vi "Build Class Hierarchy as List.vi"(8 "error in (no error)":errorcluster, 11 "List of Class Paths":path[](array[path])) -> (0 "error out":errorcluster, 3 "List of Class Paths Out":path[](array[path]))   [LabVIEW 2012, in "Palette Generation.lvlib"]
doc: "This VI builds a list of all the parent classes of the input list of class files and returns a list of all classes in the heirarachy with the base classes firts. This ensures that when we generate the palette files, the parent class root palette file will always exist and so can be linked in."
uses:
  Palette Generation.lvlib
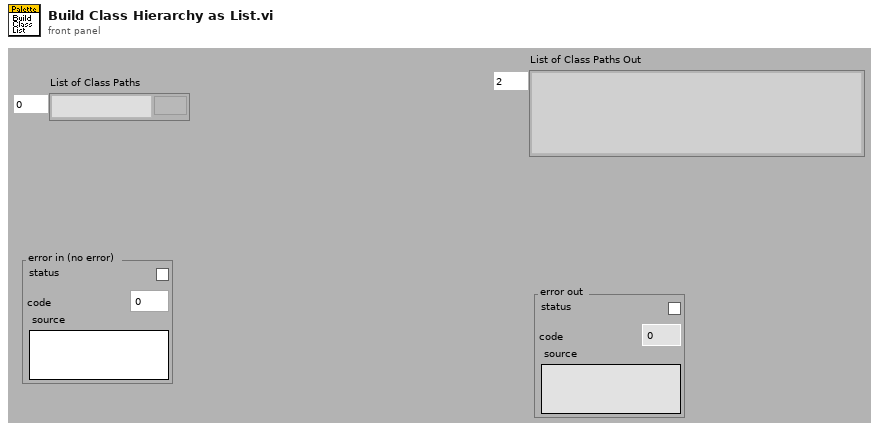
[diagram p1: front panel]
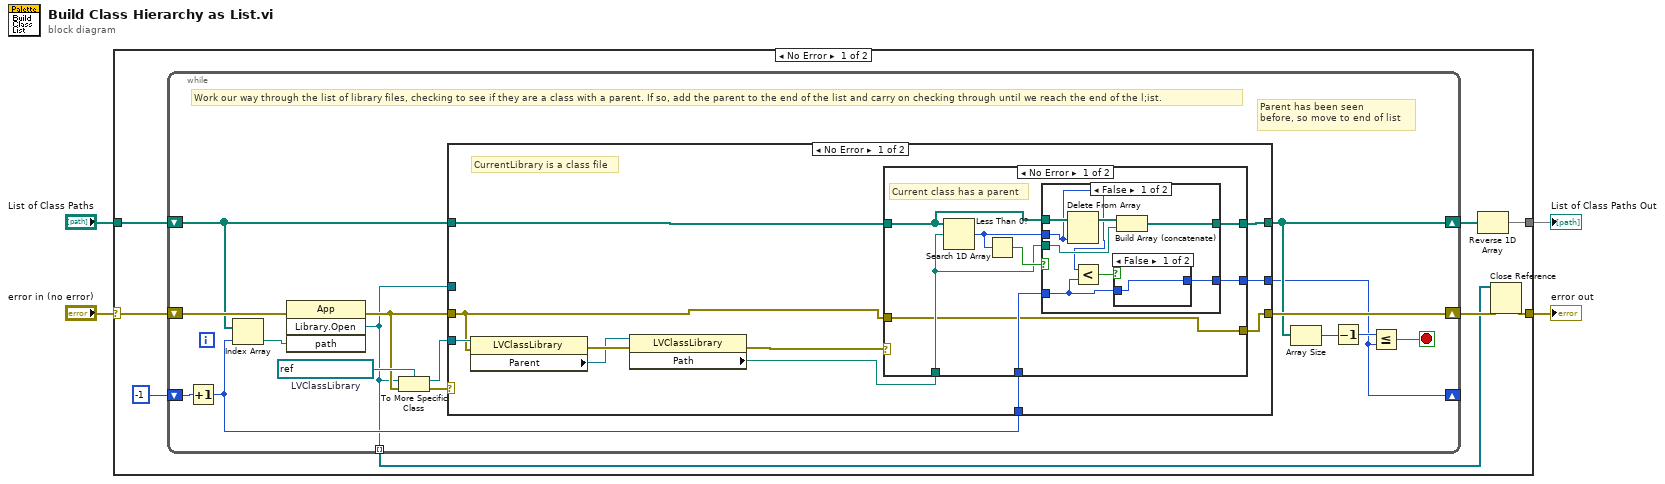
[diagram p0: block diagram]
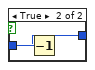
[diagram p2: hidden frame]
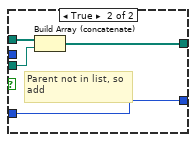
[diagram p3: hidden frame]
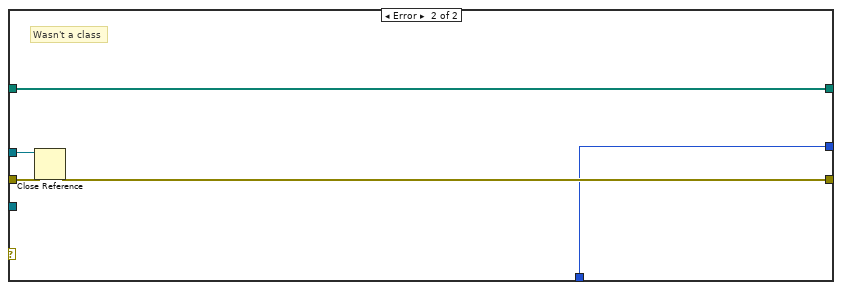
[diagram p5: hidden frame]
diagram:
  n1 = case shown="No Error" "error in (no error)" {
    selector: "error in (no error)" -> [w9 w72]
    tunnel: "List of Class Paths" -> [w12 w71]
    tunnel: [w10 w71] -> w2
    tunnel: [w5 w72] -> w1
    frame No Error {
      n2 = while {
        shift-right: [w23] -> w7
        shift-left: w9 -> [w28]
        shift-right: [w20] -> w11
        shift-left: w12 -> [w25]
        shift-right: [w14] -> _
        shift-left: -1 -> [w16]
        tunnel: [w13] -> w6 mode=indexing
        stop <- w17 stop-if-true
        w27 = refnum<vi> refnum  # LVClassLibrary
        # "Parent has been seen\nbefore, so move to end of list"
        # "Work our way through the list of library files, checking to see if they are a class with a parent. If so, add the parent to the end of the list and carry on checking through until we reach the end of the l;ist."
        n3 = Increment(x=w16) -> (x+1=w15:i32)
        n4 = Index Array(array=w25, index=w15) -> (element=w26:path)
        n5 = invoke class="App" method="Library.Open"(error in=w28, "path"=w26) -> (error out=w22:errorcluster, "Open Library"=w13:refnum<vi>)  [unwired: 2 in, 2 out]
        n6 = To More Specific Class(target class=w27, reference=w13, error in=w22) -> (specific class reference=w21:refnum<vi>, error out=w24:errorcluster)
        n7 = case shown="No Error" w24 {
          tunnel: w25 -> [w38 w70]
          tunnel: [w37 w70] -> w20
          tunnel: [w31 w67] -> w23
          tunnel: w22 -> [w29 w69]
          tunnel: w21 -> [w39 _]
          tunnel: w13 -> [_ w68]
          tunnel: [w36 w66] -> w14
          tunnel: w15 -> [w35 w66]
          frame No Error {
            # "CurrentLibrary is a class file"
            n8 = property class="LVClassLibrary"(reference=w39, error in=w29) -> (error out=w34:errorcluster, "Parent"=w33:refnum<vi>)  [unwired: 1 out]
            n9 = property class="LVClassLibrary"(reference=w33, error in=w34) -> (error out=w30:errorcluster, "Path"=w32:path)  [unwired: 1 out]
            n10 = case shown="No Error" w30 {
              tunnel: w38 -> [w46 w65]
              tunnel: [w45 w65] -> w37
              tunnel: [w43 w64] -> w36
              tunnel: w35 -> [w42 w64]
              tunnel: w32 -> [w41 _]
              tunnel: [w40 w63] -> w31
              tunnel: w29 -> [w40 w63]
              frame No Error {
                # "Current class has a parent"
                n11 = Search 1D Array(1D array=w46, element=w41) -> (index of element=w44:i32)  [unwired: 1 out]
                n12 = Less Than 0?(x=w44) -> (x < 0?=w47:bool)
                n13 = case shown="False" w47 {
                  tunnel: w46 -> [w55 w62]
                  tunnel: w41 -> [w53 w61]
                  tunnel: [w52 w60] -> w45
                  tunnel: w44 -> [w49 _]
                  tunnel: [w51 w59] -> w43
                  tunnel: w42 -> [w48 w59]
                  frame False {
                    n14 = Delete From Array(array=w55, index=w49) -> (array with subset deleted=w54:path[])  [unwired: 1 in, 1 out]
                    n15 = Less?(x=w49, y=w48) -> (x < y?=w50:bool)
                    n16 = case shown="False" w50 {
                      tunnel: w48 -> [w56 w58]
                      tunnel: [w56 w57] -> w51
                      frame False {
                      }
                      frame True {
                        n17 = Decrement(x=w58) -> (x-1=w57:i32)
                      }
                    }
                    n18 = Build Array (concatenate)(w54, w53) -> (w52:path[])
                  }
                  frame True {
                    # "Parent not in list, so\nadd"
                    n19 = Build Array (concatenate)(w62, w61) -> (w60:path[])
                  }
                }
              }
              frame Error {
                # "Class parent path was bad - this means this was a base class"
              }
            }
          }
          frame Error {
            # "Wasn't a class"
            n20 = Close Reference(reference=w68, error in (no error)=w69) -> (error out=w67:errorcluster)
          }
        }
        n21 = Array Size(array=w20) -> (size(s)=w19:i32)
        n22 = Decrement(x=w19) -> (x-1=w18:i32)
        n23 = Less Or Equal?(x=w18, y=w14) -> (x <= y?=w17:bool)
      }
      n24 = Reverse 1D Array(array=w11) -> (reversed array=w10:path[])
      n25 = Close Reference(reference=w6, error in (no error)=w7) -> (error out=w5:errorcluster)
    }
    frame Error {
    }
  }
  "List of Class Paths Out" <- w2
  "error out" <- w1
